vi "New Toast Notification.vi"(8 "error in":errorcluster, 11 "XML Document in":refnum<k24>) -> (0 "error out":errorcluster, 2 "Toast Notification":refnum<k24>, 3 "XML Document out":refnum<k24>)   [LabVIEW 2026, in "ToastNotification.lvlib" / "Toast Native.lvlib"]
doc: "Construct Windows.UI.Notifications.ToastNotification from a borrowed WinRT XML Document through runtime reflection. Skipped on incoming error. Caller owns Toast Notification and still owns XML Document; neither is closed here. Release the temporary Type even on failure. Does not display the toast."
uses:
  Toast Native.lvlib
  Reflection DotNet/Reflection DotNet.lvlib
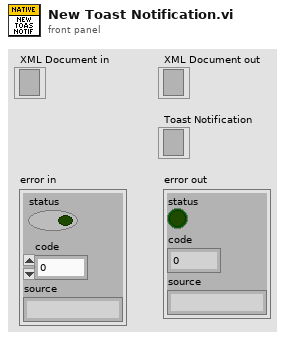
[diagram p1: front panel]
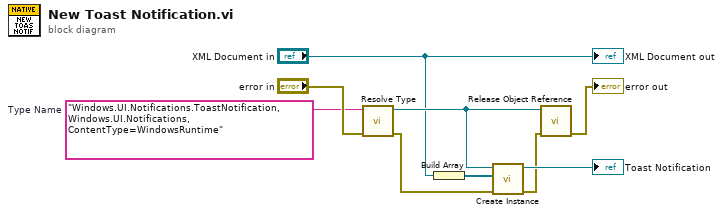
[diagram p0: block diagram]
diagram:
  w8 = "Windows.UI.Notifications.ToastNotification, Windows.UI.Notifications, ContentType=WindowsRuntime"  # Type Name
  n1 = call "Resolve Type.vi"("error in"="error in", "Type Name"=w8) -> ("error out"=w7:errorcluster, "Runtime Type"=w5:refnum<k24>)  [unwired: 8 in]
  n2 = Build Array("XML Document in") -> (w6:refnum<k24>[])
  n3 = call "Create Instance.vi"("error in"=w7, "parameters"=w6, "Runtime Type"=w5) -> ("error out"=w2:errorcluster, "Instance"=→"Toast Notification":refnum<k24>)  [unwired: 7 in]
  n4 = call "Release Object Reference.vi"("error in"=w2, "object"=w5) -> ("error out"=→"error out":errorcluster)  [unwired: 9 in]
  "XML Document out" <- "XML Document in"
